vi "libssh2_userauth_hostbased_fromfile_ex.vi"(4 "local_username":string, 5 "private key":path, 6 "hostname":string, 7 "public key":path, 8 "error in (no error)":errorcluster, 9 "passphrase":string, 10 "username":string, 11 "session":T1) -> (0 "error out":errorcluster)   [LabVIEW 2017, in "libssh2.lvlib"]
doc: "Authenticate a session using host-based authentication with a public key file."
uses:
  libssh2.lvlib
  Session Refnum.ctl
  Not A Session.vi
  <vilib>/Utility/error.llb/Error Cluster From Error Code.vi
  Global Settings.vi
  Read Session Refnum.vi
  <vilib>/Utility/semaphor.llb/Acquire Semaphore.vi
  <vilib>/Utility/semaphor.llb/Release Semaphore.vi
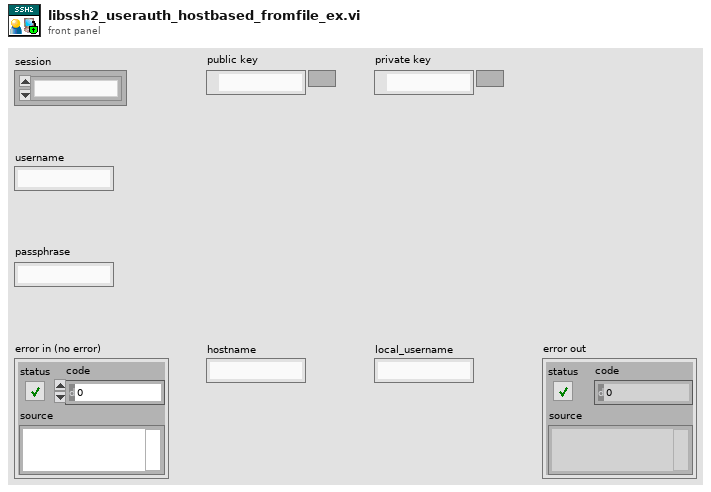
[diagram p1: front panel]
types:
  T1 = typedef "libssh2.lvlib/Session Refnum.ctl" = refnum<k1>
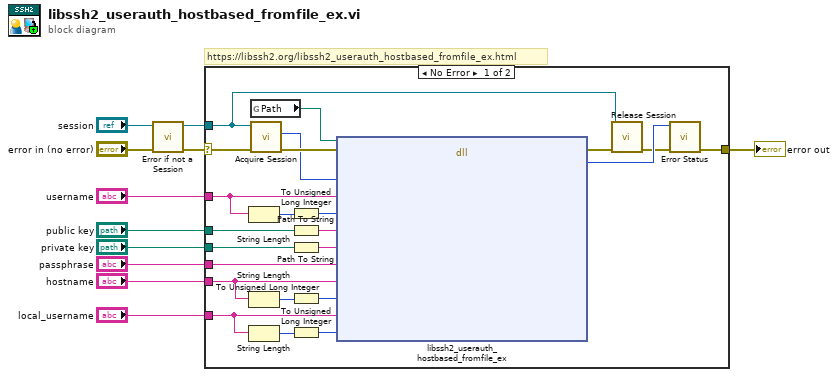
[diagram p0: block diagram]
diagram:
  # "https://libssh2.org/libssh2_userauth_hostbased_fromfile_ex.html"
  n1 = call "Error if not a Session.vi"("error in (no error)"="error in (no error)", "session"="session") -> ("error out"=w8:errorcluster, "session out"=w6:T1)  [unwired: 8 in]
  n2 = case shown="No Error" w8 {
    selector: w8 -> [w33 w35]
    tunnel: "username" -> [w34 _]
    tunnel: [w32 w35] -> w10
    tunnel: w6 -> [w12 _]
    tunnel: "public key" -> [w24 _]
    tunnel: "private key" -> [w23 _]
    tunnel: "passphrase" -> [w22 _]
    tunnel: "hostname" -> [w15 _]
    tunnel: "local_username" -> [w14 _]
    frame No Error {
      n3 = String Length(string=w34) -> (length=w29:i32)
      n4 = String Length(string=w15) -> (length=w19:i32)
      n5 = String Length(string=w14) -> (length=w18:i32)
      n6 = global read "Global Settings.vi" "Path"() -> (w26:path)
      n7 = call "Acquire Session.vi"("error in (no error)"=w33, "session"=w12) -> ("error out"=w28:errorcluster, "LIBSSH2_SESSION*"=w27:u64)  [unwired: 7 in, 1 out]
      n8 = To Unsigned Long Integer(number=w29) -> (unsigned 32bit integer=w31:u32)
      n9 = Path To String(path=w24) -> (string=w21:string)
      n10 = Path To String(path=w23) -> (string=w20:string)
      n11 = To Unsigned Long Integer(number=w19) -> (unsigned 32bit integer=w16:u32)
      n12 = To Unsigned Long Integer(number=w18) -> (unsigned 32bit integer=w17:u32)
      n13 = dll-call lib="?" fn="libssh2_userauth_hostbased_fromfile_ex"(path in=w26, error in=w28, "session"=w27, "username"=w34, "username_len"=w31, "publickey"=w21, "privatekey"=w20, "passphrase"=w22, "hostname"=w15, "hostname_len"=w16, "local_username"=w14, "local_username_len"=w17) -> (error out=w30:errorcluster, "return value"=w25:i32)  [unwired: 11 in, 1 out]
      n14 = call "Release Session.vi"("error in (no error)"=w30, "session"=w12) -> ("error out"=w13:errorcluster)  [unwired: 9 in]
      n15 = call "Error Status.vi"("error in (no error)"=w13, "return value"=w25) -> ("error out"=w32:errorcluster)  [unwired: 8 in, 1 out]
    }
    frame Error {
    }
  }
  "error out" <- w10
